vi "round OBW Measurement.vi"(8 "error in (no error)":errorcluster, 10 "OBW Measurement Raw Result":dbl[](array[numeric]), 11 "Keysight 9020A in":refnum<class "Keysight 9020A.lvclass">) -> (0 "error out":errorcluster, 2 "OBW Measurement Rounded Result":dbl[](array[numeric]), 3 "Keysight 9020A out":refnum<class "Keysight 9020A.lvclass">)   [LabVIEW 2023, in "Spectrum Analyzer.lvlib" / "Keysight 9020A.lvclass"]
uses:
  Keysight 9020A.lvclass
  Keysight 9020A.lvclass/Keysight 9020A.ctl
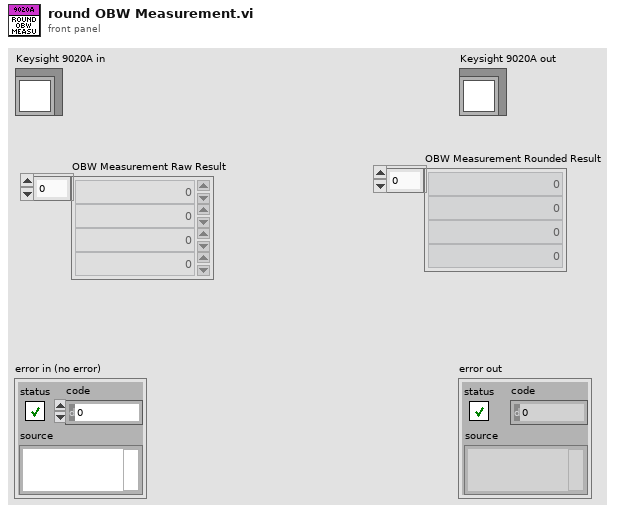
[diagram p1: front panel]
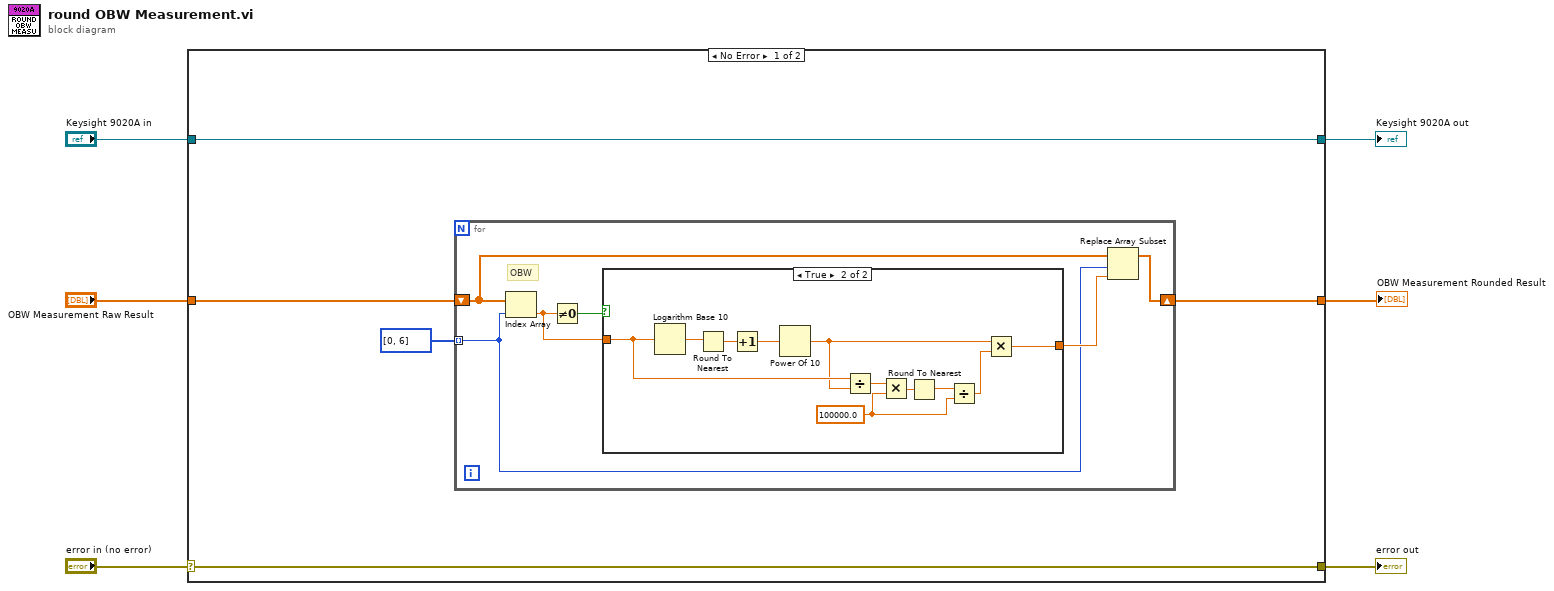
[diagram p0: block diagram]
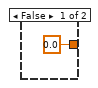
[diagram p2: hidden frame]
diagram:
  n1 = case shown="No Error" "error in (no error)" {
    selector: "error in (no error)" -> [w11 w31]
    tunnel: [w11 w31] -> w5
    tunnel: [w10 w30] -> w3
    tunnel: "Keysight 9020A in" -> [w10 w30]
    tunnel: "OBW Measurement Raw Result" -> [w9 _]
    tunnel: [w8 _] -> w1
    frame No Error {
      n2 = for {
        shift-right: [w13] -> w8
        shift-left: w9 -> [w14]
        tunnel: i32[] [0, 6] ("index") -> [w12] mode=indexing
        # "OBW"
        n3 = Index Array(array=w14, index=w12) -> (element=w17:dbl)
        n4 = Not Equal To 0?(x=w17) -> (x != 0?=w16:bool)
        n5 = case shown="True" w16 {
          tunnel: w17 -> [_ w26]
          tunnel: [0.0 w19] -> w15
          frame False {
          }
          frame True {
            w21 = 100000.0 ("y")
            n6 = Logarithm Base 10(1:w26) -> (0:w28:dbl)
            n7 = Round To Nearest(number=w28) -> (nearest integer value=w29:dbl)
            n8 = Increment(x=w29) -> (x+1=w27:dbl)
            n9 = Power Of 10(x=w27) -> (10^x=w23:dbl)
            n10 = Divide(x=w26, y=w23) -> (x/y=w25:dbl)
            n11 = Multiply(x=w25, y=w21) -> (x*y=w24:dbl)
            n12 = Round To Nearest(number=w24) -> (nearest integer value=w22:dbl)
            n13 = Divide(x=w22, y=w21) -> (x/y=w20:dbl)
            n14 = Multiply(x=w23, y=w20) -> (x*y=w19:dbl)
          }
        }
        n15 = Replace Array Subset(array=w14, new element=w15, index=w12) -> (w13:dbl[])
      }
    }
    frame Error {
    }
  }
  "error out" <- w5
  "Keysight 9020A out" <- w3
  "OBW Measurement Rounded Result" <- w1
